vi "RDC-get_specific_data_points.vi"(10 "Requested Frequencies":dbl[](array[numeric])=[300000000.0, 600000000.0, 1000000000.0, 3000000000.0], 11 "Element map":map{dbl, T1}(c390)) -> (1 "Data points":T1[](array[typedef]), 2 "Actual Frequencies":dbl[](array[numeric]))   [LabVIEW 2020, in "RDC-Reflection_Data_Computation.lvlib"]
doc: "Looks up the requested frequencies in an element map and returns the matching data points and their actual frequencies."
uses:
  RDC-Reflection_Data_Computation.lvlib
  Reflector/RFH-common_data_format_element.ctl
  Reflector/RFH-Reflection_File_Handler.lvlib
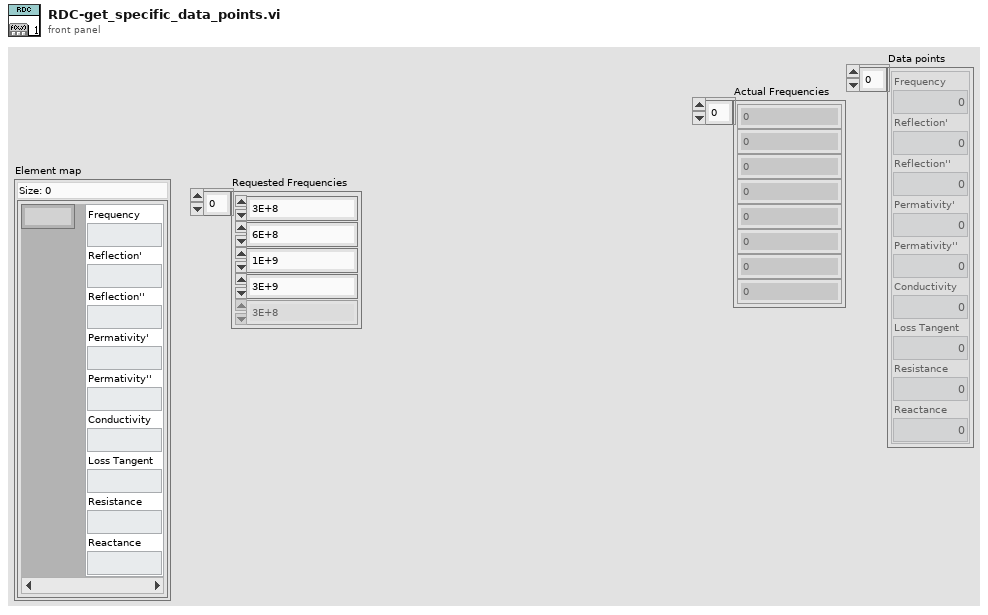
[diagram p1: front panel]
types:
  T1 = typedef "RFH-Reflection_File_Handler.lvlib/RFH-common_data_format_element.ctl" = cluster{"Frequency":dbl, "Reflection'":dbl, "Reflection''":dbl, "Permativity'":dbl, "Permativity''":dbl, "Conductivity":dbl, "Loss Tangent":dbl, "Resistance":dbl, "Reactance":dbl}
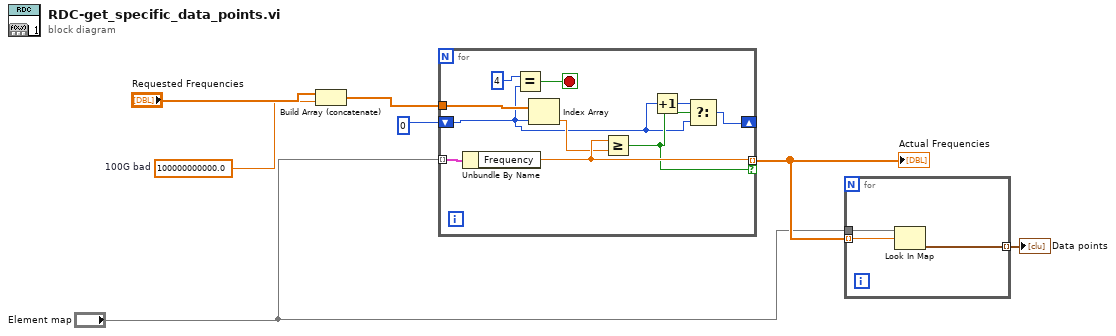
[diagram p0: block diagram]
diagram:
  w4 = 100000000000.0  # 100G bad
  n1 = Build Array (concatenate)("Requested Frequencies", w4) -> (w6:dbl[])
  n2 = for {
    tunnel: "Element map" -> [w17] mode=indexing
    tunnel: [w14] -> w3 mode=indexing if=w12
    tunnel: w6 -> [w16]
    shift-right: [w9] -> _
    shift-left: 0 ("index") -> [w10]
    stop <- w15 stop-if-true
    n3 = Unbundle By Name(w17) -> ("Frequency"=w14:dbl)
    n4 = Equal?(x=4 ("y"), y=w10) -> (x = y?=w15:bool)
    n5 = Index Array(array=w16, index=w10) -> (element=w13:dbl)
    n6 = Greater Or Equal?(x=w14, y=w13) -> (x >= y?=w12:bool)
    n7 = Increment(x=w10) -> (x+1=w11:i32)
    n8 = Select(t=w11, s=w12, f=w10) -> (s? t:f=w9:i32)
  }
  "Actual Frequencies" <- w3
  n9 = for {
    tunnel: w3 -> [w19] mode=indexing
    tunnel: "Element map" -> [w20]
    tunnel: [w18] -> w1 mode=indexing
    n10 = Look In Map(map=w20, key=w19) -> (value=w18:T1)  [unwired: 1 in, 1 out]
  }
  "Data points" <- w1
